vi "Preset_Edit.vi"() -> ()   [LabVIEW 2020, in "Sgraph_lib_V1.lvlib" / "Gviewer.lvclass"]
doc: "Andre Koelewijn, 20 jan 2021\n\nEdit TAGs to display"
uses:
  Gviewer.lvclass
  controls/EditTagOneTag.ctl
  controls/Typedef_Gserver-Replies.ctl
  controls/Typedef_ServerActions.ctl
  DBAL/controls/DBAL_TAGprops.ctl
  DBAL/controls/DBAL_TAGpropEdit.ctl
  Common/controls/typedef_com_TagProp.ctl
  <vilib>/Utility/miscctls.llb/LVPointTypeDef.ctl
  Builds/Sgraph_lib_V1.lvlib
panel:
  in  "PresetPath":path
  in  "PresetName":string
  in  "SaveTime":bool
  in  "OK":bool
  out "tag-info":string
  in  "SaveAs":bool
  in  "Save":bool
  in  "Cancel":bool
  in  "Selector":i32[](listbox)
  in  "Presets":T1[](array[typedef]) {"max" format="%#_3p"; "min" format="%#_3p"}
  in  "Exit_event":bool
  in  "TAGproperties":T2 {"TAGprop"."TagFunc" format="%08x"; "TAGprop"."RangeL" format="%.2f"; "TAGprop"."RangeH" format="%.2f"}
  in  "GViewer-Queue":refnum<queue>
  # "Tag name"
  # "scale L"
  # "scale H"
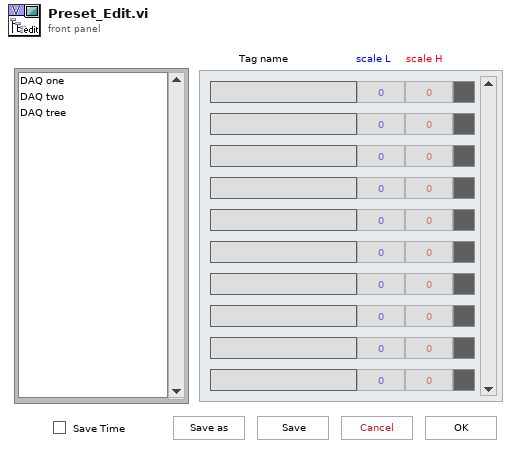
[diagram p1: front panel]
types:
  T1 = typedef "Sgraph_lib_V1.lvlib/Gviewer.lvclass/EditTagOneTag.ctl" = cluster{"TAG":string, "min":dbl, "max":dbl, "Color":u32}
  T2 = typedef "Sgraph_lib_V1.lvlib/DBAL_TAGprops.ctl" = T3[]
  T3 = typedef "Sgraph_lib_V1.lvlib/DBAL_TAGpropEdit.ctl" = cluster{"TAG":string, "Qtype":string, "TAGprop":T4}
  T4 = typedef "Sgraph_lib_V1.lvlib/typedef_com_TagProp.ctl" = cluster{"Description":string, "EngUnits":string, "RangeH":dbl, "RangeL":dbl, "Resolution":i32, "Obsolete":bool, "ChangeDate":timestamp, "ChangeSource":string, "ChangeReason":string, "TagFunc":u32}
  T5 = typedef "LVPointTypeDef.ctl" = cluster{"Horizontal":i16, "Vertical":i16}
  T6 = typedef "Sgraph_lib_V1.lvlib/Typedef_ServerActions.ctl" = enum16{"GraphUpdate", "SendAllTags", "SendIniPath", "SetGeneralOptions", "EditTagsOpen", "EditTagsPresetSave", "EditTagsPresetLoad", "EditTagsClose", "NewTagSelection", "ExitGraph"}
  T7 = typedef "Typedef_Gserver-Replies.ctl" = cluster{"ServerActions":T6, "data":variant, "Source":string, "Time Stamp":timestamp}
  T8 = enum32{"Invalid", "Standard", "Closed", "Hidden", "Minimized", "Maximized"}
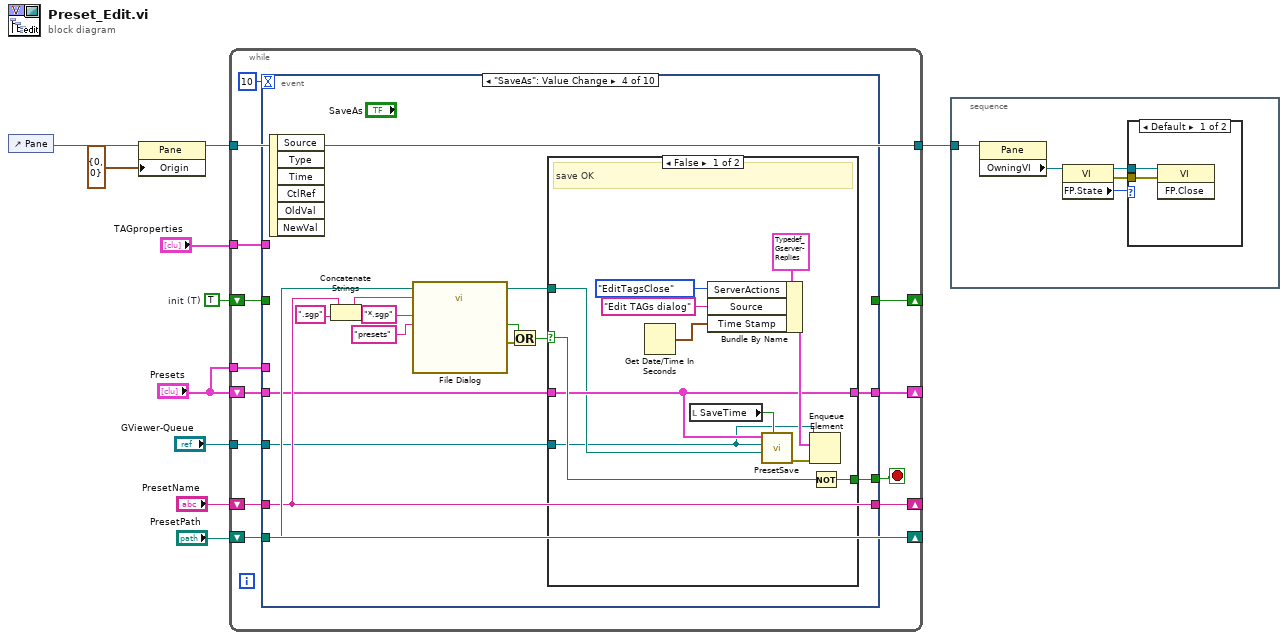
[diagram p0: block diagram]
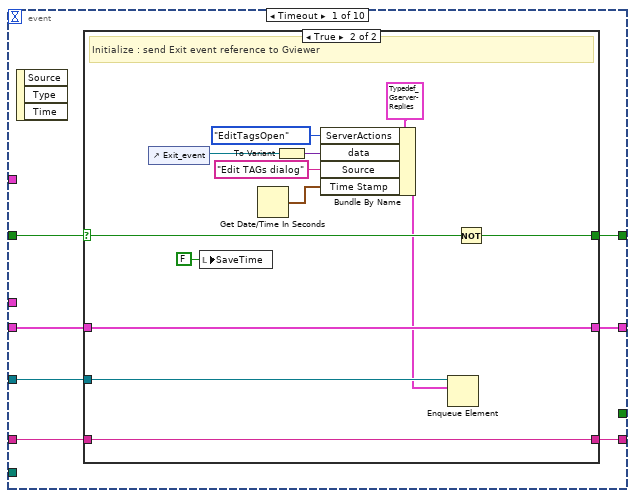
[diagram p3: hidden frame]
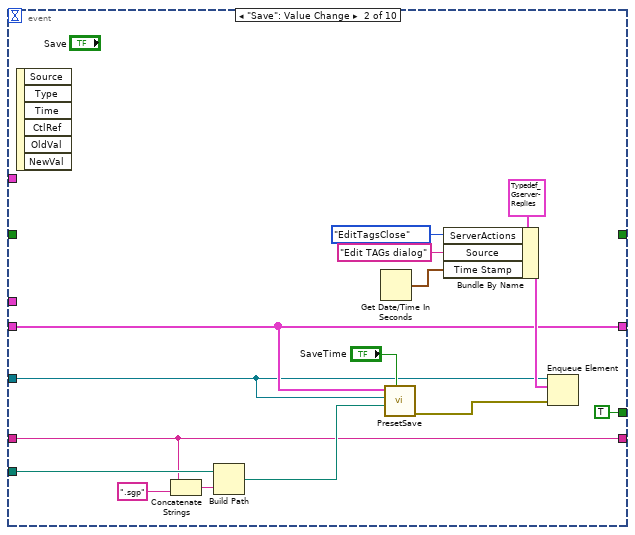
[diagram p5: hidden frame]
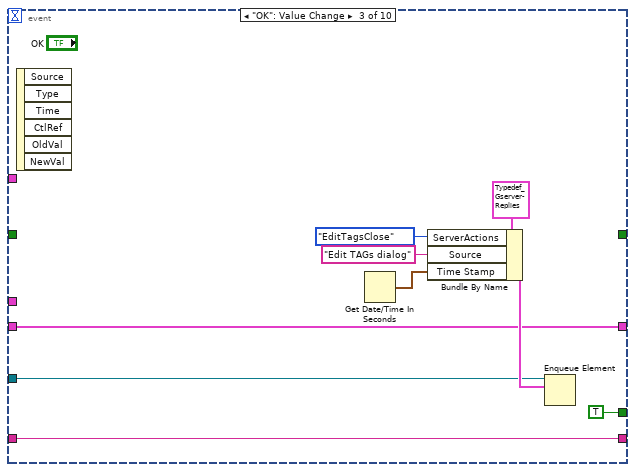
[diagram p6: hidden frame]
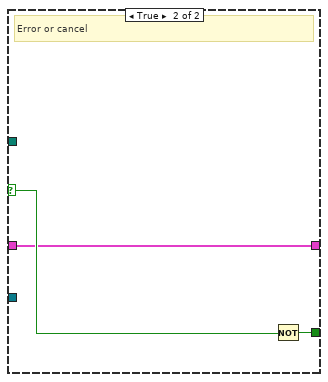
[diagram p7: hidden frame]
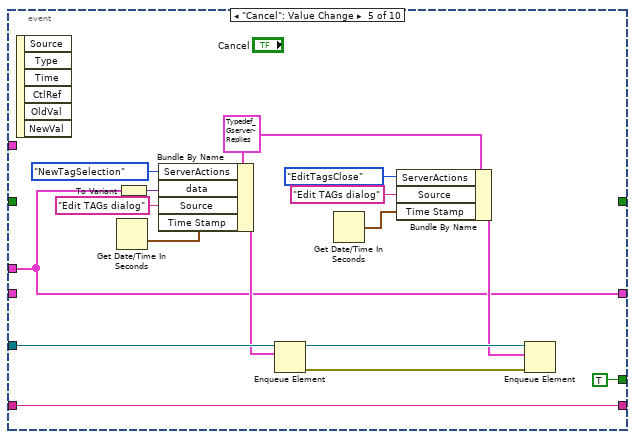
[diagram p8: hidden frame]
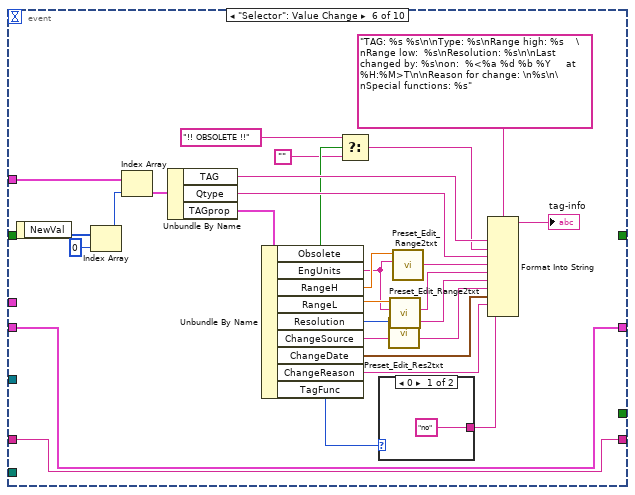
[diagram p9: hidden frame]
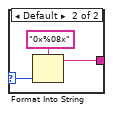
[diagram p10: hidden frame]
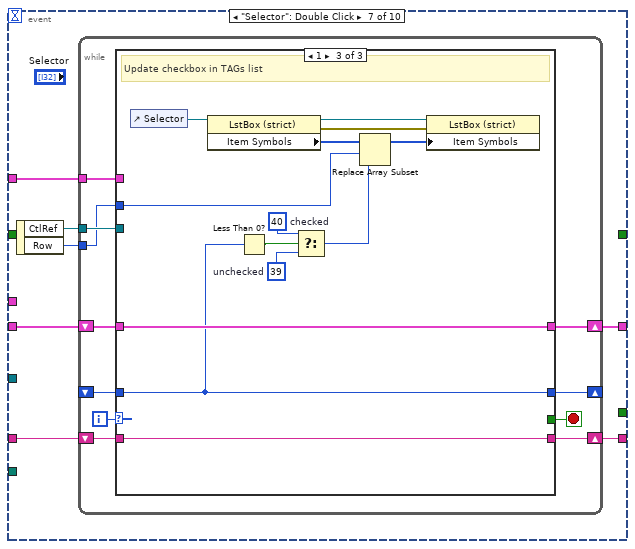
[diagram p11: hidden frame]
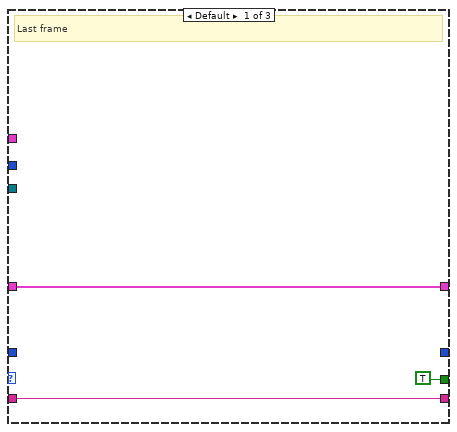
[diagram p12: hidden frame]
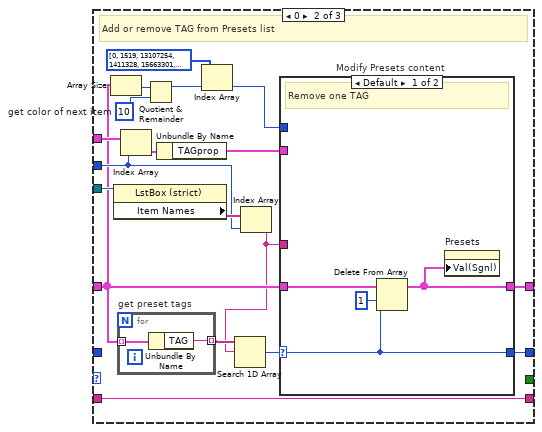
[diagram p13: hidden frame]
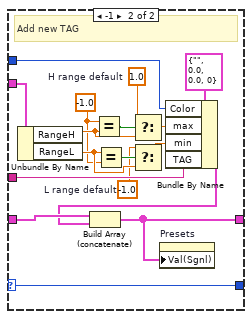
[diagram p14: hidden frame]
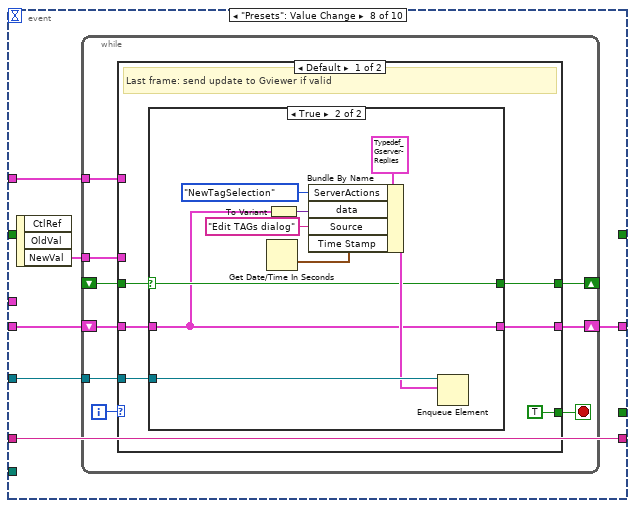
[diagram p15: hidden frame]
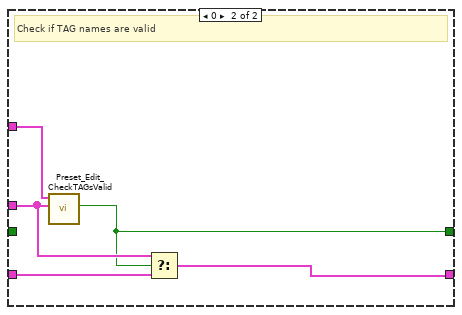
[diagram p17: hidden frame]
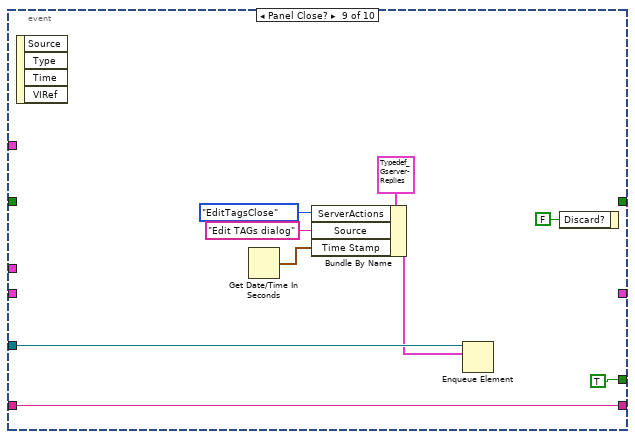
[diagram p18: hidden frame]
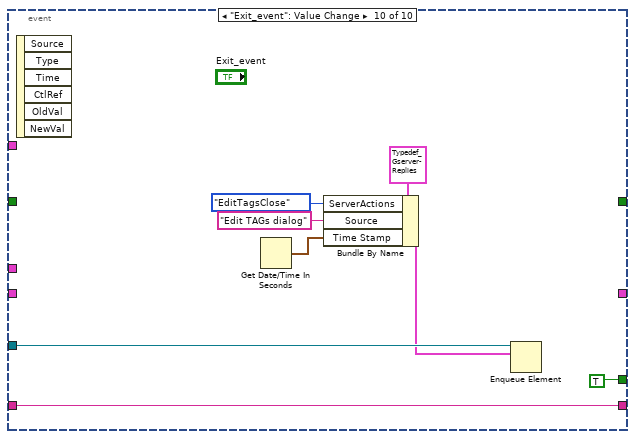
[diagram p19: hidden frame]
diagram:
  w5 = TRUE  # init (T)
  n1 = control-ref of="Pane"() -> (w9:refnum<vi>)
  n2 = property class="Pane"(reference=w9, "Origin"=T5 {"Horizontal"=0, "Vertical"=0}) -> (reference out=w8:refnum<vi>)  [unwired: 1 in, 1 out]
  n3 = while {
    tunnel: w8 -> [w14]
    tunnel: "TAGproperties" -> [w21]
    tunnel: "GViewer-Queue" -> [w18]
    shift-right: [w19] -> _
    shift-left: "Presets" -> [w20]
    shift-right: [w16] -> _
    shift-left: w5 -> [w17]
    tunnel: "Presets" -> [w15]
    tunnel: [w14] -> w3
    shift-right: [w12] -> _
    shift-left: "PresetName" -> [w13]
    shift-right: [w11] -> _
    shift-left: "PresetPath" -> [w11]
    stop <- w23 stop-if-true
    n4 = event shown="[3] \"SaveAs\": Value Change" {
      selector: _ -> [_ _ _ _ _ _ _ _ _ _]
      dyn-events: _ -> [_ _ _ _ _ _ _ _ _ _]
      timeout: 10 -> [_ _ _ _ _ _ _ _ _ _]
      tunnel: [_ TRUE TRUE w75 TRUE _ _ _ TRUE TRUE] -> w23
      tunnel: w21 -> [_ _ _ _ _ w143 w150 w224 _ _]
      tunnel: w20 -> [w29 w51 w64 w73 _ w117 w152 w228 _ _]
      tunnel: [w28 w51 w64 w72 w102 w117 w151 w227 _ _] -> w19
      tunnel: w18 -> [w26 w50 w62 w71 w111 _ _ w226 w262 w275]
      tunnel: w17 -> [w30 _ _ _ _ _ _ _ _ _]
      tunnel: [w27 _ _ _ _ _ _ _ _ _] -> w16
      tunnel: w15 -> [_ _ _ _ w102 _ _ _ _ _]
      tunnel: w13 -> [w25 w48 w63 w81 w100 w116 w149 w223 w260 w269]
      tunnel: [w24 w48 w63 w81 w100 w116 w148 w223 w260 w269] -> w12
      tunnel: w11 -> [_ w49 _ w84 _ _ _ _ _ _]
      event Timeout {
        n5 = event-data() -> ()  [unwired: 1 in, 3 out]
        n6 = case shown="True" w30 {
          selector: w30 -> [w32 w45]
          tunnel: w29 -> [w33 w46]
          tunnel: [w33 w46] -> w28
          tunnel: [w32 w44] -> w27
          tunnel: w26 -> [_ w43]
          tunnel: w25 -> [w31 w34]
          tunnel: [w31 w34] -> w24
          frame False {
            # "normal idle operation"
          }
          frame True {
            # "Initialize : send Exit event reference to Gviewer"
            n7 = control-ref of="Exit_event"() -> (w40:refnum<vi>)
            n8 = local write "SaveTime"(FALSE ("TimeToo")) -> ()
            n9 = Get Date/Time In Seconds() -> (seconds since 1Jan1904=w37:timestamp)
            n10 = To Variant(anything=w40) -> (Variant=w39:variant)
            n11 = Bundle By Name(cluster=T7 {"ServerActions"=enum."GraphUpdate", "data"=variant, "Source"="", "Time Stamp"=timestamp(0 s since 1904-01-01)} ("element"), "ServerActions"=Typedef_ServerActions."EditTagsOpen", "data"=w39, "Source"="Edit TAGs dialog", "Time Stamp"=w37) -> (w36:T7)
            n12 = Enqueue Element(queue=w43, element=w36) -> ()  [unwired: 2 in, 3 out]
            n13 = Not(x=w45) -> (.not. x?=w44:bool)
          }
        }
      }
      event "Save": Value Change {
        n14 = event-data() -> ()  [unwired: 1 in, 6 out]
        n15 = Concatenate Strings(w48, ".sgp" ("string")) -> (w55:string)
        n16 = Build Path(base path=w49, name or relative path=w55) -> (appended path=w54:path)
        n17 = Get Date/Time In Seconds() -> (seconds since 1Jan1904=w61:timestamp)
        n18 = call "PresetSave.vi"("Save time?"="SaveTime", "PresetFilePath"=w54, "GViewer-Queue"=w50, "Presets"=w51) -> ("error out"=w47:errorcluster)  [unwired: 7 in]
        n19 = Bundle By Name(cluster=T7 {"ServerActions"=enum."GraphUpdate", "data"=variant, "Source"="", "Time Stamp"=timestamp(0 s since 1904-01-01)} ("element"), "ServerActions"=Typedef_ServerActions."EditTagsClose", "Source"="Edit TAGs dialog", "Time Stamp"=w61) -> (w60:T7)
        n20 = Enqueue Element(queue=w50, element=w60, error in (no error)=w47) -> ()  [unwired: 1 in, 3 out]
      }
      event "OK": Value Change {
        n21 = event-data() -> ()  [unwired: 1 in, 6 out]
        n22 = Get Date/Time In Seconds() -> (seconds since 1Jan1904=w70:timestamp)
        n23 = Bundle By Name(cluster=T7 {"ServerActions"=enum."GraphUpdate", "data"=variant, "Source"="", "Time Stamp"=timestamp(0 s since 1904-01-01)} ("element"), "ServerActions"=Typedef_ServerActions."EditTagsClose", "Source"="Edit TAGs dialog", "Time Stamp"=w70) -> (w66:T7)
        n24 = Enqueue Element(queue=w62, element=w66) -> ()  [unwired: 2 in, 3 out]
      }
      event "SaveAs": Value Change {
        n25 = event-data() -> ()  [unwired: 1 in, 6 out]
        n26 = Concatenate Strings(w81, ".sgp" ("string")) -> (w80:string)
        n27 = call "File Dialog"("start path"=w84, "default name"=w80, "pattern (all files)"="*.sgp" ("string"), "pattern label"="presets") -> ("selected path"=w74:path, "cancelled"=w77:bool, "error out"=w78:errorcluster)  [unwired: 8 in, 1 out]
        n28 = Or(x=w77, y=w78) -> (x .or. y?=w76:bool)
        n29 = case shown="False" w76 {
          selector: w76 -> [w96 w99]
          tunnel: [w95 w98] -> w75
          tunnel: w74 -> [w86 _]
          tunnel: w73 -> [w87 w97]
          tunnel: [w87 w97] -> w72
          tunnel: w71 -> [w85 _]
          frame False {
            # "save OK"
            n30 = Get Date/Time In Seconds() -> (seconds since 1Jan1904=w93:timestamp)
            n31 = local read "SaveTime"() -> (w91:bool)
            n32 = Bundle By Name(cluster=T7 {"ServerActions"=enum."GraphUpdate", "data"=variant, "Source"="", "Time Stamp"=timestamp(0 s since 1904-01-01)} ("element"), "ServerActions"=Typedef_ServerActions."EditTagsClose", "Source"="Edit TAGs dialog", "Time Stamp"=w93) -> (w94:T7)
            n33 = call "PresetSave.vi"("Save time?"=w91, "PresetFilePath"=w86, "GViewer-Queue"=w85, "Presets"=w87) -> ("error out"=w92:errorcluster)  [unwired: 7 in]
            n34 = Enqueue Element(queue=w85, element=w94, error in (no error)=w92) -> ()  [unwired: 1 in, 3 out]
            n35 = Not(x=w96) -> (.not. x?=w95:bool)
          }
          frame True {
            # "Error or cancel"
            n36 = Not(x=w99) -> (.not. x?=w98:bool)
          }
        }
      }
      event "Cancel": Value Change {
        w106 = T7 {"ServerActions"=enum."GraphUpdate", "data"=variant, "Source"="", "Time Stamp"=timestamp(0 s since 1904-01-01)} ("element")
        n37 = event-data() -> ()  [unwired: 1 in, 6 out]
        n38 = Get Date/Time In Seconds() -> (seconds since 1Jan1904=w115:timestamp)
        n39 = To Variant(anything=w102) -> (Variant=w114:variant)
        n40 = Bundle By Name(cluster=w106, "ServerActions"=Typedef_ServerActions."NewTagSelection", "data"=w114, "Source"="Edit TAGs dialog", "Time Stamp"=w115) -> (w110:T7)
        n41 = Enqueue Element(queue=w111, element=w110) -> (queue out=w104:refnum<queue>, error out=w105:errorcluster)  [unwired: 2 in, 1 out]
        n42 = Get Date/Time In Seconds() -> (seconds since 1Jan1904=w109:timestamp)
        n43 = Bundle By Name(cluster=w106, "ServerActions"=Typedef_ServerActions."EditTagsClose", "Source"="Edit TAGs dialog", "Time Stamp"=w109) -> (w103:T7)
        n44 = Enqueue Element(queue=w104, element=w103, error in (no error)=w105) -> ()  [unwired: 1 in, 3 out]
      }
      event "Selector": Value Change {
        n45 = event-data() -> ("NewVal"=w142:i32[])  [unwired: 1 in]
        n46 = Index Array(array=w142, index=0) -> (element=w140:i32)
        n47 = Index Array(array=w143, index=w140) -> (element=w139:T3)
        n48 = Unbundle By Name(w139) -> ("TAG"=w130:string, "Qtype"=w136:string, "TAGprop"=w138:T4)
        n49 = Unbundle By Name(w138) -> ("Obsolete"=w129:bool, "EngUnits"=w123:string, "RangeH"=w125:dbl, "RangeL"=w124:dbl, "Resolution"=w121:i32, "ChangeSource"=w135:string, "ChangeDate"=w134:timestamp, "ChangeReason"=w133:string, "TagFunc"=w119:u32)
        n50 = Select(t="!! OBSOLETE !!" ("format string"), s=w129, f="") -> (s? t:f=w128:string)
        n51 = case shown="0" w119 {
          selector: w119 -> [_ w146]
          tunnel: ["no" w145] -> w118
          frame 0 {
          }
          frame Default {
            n52 = Format Into String(format string="0x%08x", w146) -> (resulting string=w145:string)  [unwired: 2 in, 1 out]
          }
        }
        n53 = call "Preset_Edit_Res2txt.vi"("Resolution"=w121) -> ("Resolution text"=w120:string)  [unwired: 10 in]
        n54 = call "Preset_Edit_Range2txt.vi"("Engineering units"=w123, "Range"=w124) -> ("RangeInfo"=w122:string)  [unwired: 9 in]
        n55 = call "Preset_Edit_Range2txt.vi"("Engineering units"=w123, "Range"=w125) -> ("RangeInfo"=w126:string)  [unwired: 9 in]
        n56 = Format Into String(format string="TAG: %s %s\n\nType: %s\nRange high: %s    \nRange low:  %s\nResolution: %s\n\nLast changed by: %s\non:  %<%a %d %b %Y     at  %H:%M>T\n\nReason for change: \n%s\n\nSpecial functions: %s", w130, w128, w136, w126, w122, w120, w135, w134, w133, w118) -> (resulting string=→"tag-info":string)  [unwired: 2 in, 1 out]
      }
      event "Selector": Double Click {
        n57 = event-data() -> ("CtlRef"=w154:refnum<vi>, "Row"=w153:i32)  [unwired: 1 in]
        n58 = while {
          tunnel: w154 -> [w161]
          tunnel: w153 -> [w160]
          shift-right: [w163] -> w151
          shift-left: w152 -> [w164]
          tunnel: w150 -> [w162]
          shift-right: [w159] -> _
          shift-left: _ -> [w158]
          shift-right: [w155] -> w148
          shift-left: w149 -> [w156]
          i -> [w165]
          stop <- w157 stop-if-true
          n59 = case shown="1" w165 {
            tunnel: w164 -> [w167 w175 w216]
            tunnel: [w167 w173 w216] -> w163
            tunnel: w162 -> [_ w179 _]
            tunnel: w161 -> [_ w180 _]
            tunnel: w160 -> [_ w178 w217]
            tunnel: [_ w170 w215] -> w159
            tunnel: w158 -> [_ _ w215]
            tunnel: [TRUE _ _] -> w157
            tunnel: w156 -> [w166 w169 w210]
            tunnel: [w166 w169 w210] -> w155
            frame Default {
              # "Last frame"
            }
            frame 0 {
              w185 = 10  # get color of next item
              # "Add or remove TAG from Presets list"
              n60 = Array Size(array=w175) -> (size(s)=w186:i32)
              n61 = property class="LstBox (strict)"(reference=w180) -> ("Item Names"=w182:string[])  [unwired: 1 in, 2 out]
              n62 = for "get preset tags" {
                tunnel: w175 -> [w209] mode=indexing
                tunnel: [w208] -> w177 mode=indexing
                n63 = Unbundle By Name(w209) -> ("TAG"=w208:string)
              }
              n64 = Index Array(array=w179, index=w178) -> (element=w181:T3)
              n65 = Quotient & Remainder(x=w186, y=w185) -> (x-y*floor(x/y)=w183:i32)  [unwired: 1 out]
              n66 = Unbundle By Name(w181) -> ("TAGprop"=w172:T4)
              n67 = Index Array(array=u32[] [0, 1519, 13107254, 1411328, 15663301, 14444288, 40861, 6375227, 6783580, 10450432], index=w183) -> (element=w174:u32)
              n68 = Index Array(array=w182, index=w178) -> (element=w171:string)
              n69 = Search 1D Array(1D array=w177, element=w171) -> (index of element=w176:i32)  [unwired: 1 in]
              n70 = case "Modify Presets content" shown="Default" w176 {
                selector: w176 -> [w188 w192]
                tunnel: [w187 w191] -> w173
                tunnel: w175 -> [w189 w205]
                tunnel: w174 -> [_ w206]
                tunnel: w172 -> [_ w197]
                tunnel: w171 -> [_ w194]
                tunnel: [w188 w192] -> w170
                frame Default {
                  # "Remove one TAG"
                  n71 = Delete From Array(array=w189, length=1, index=w188) -> (array with subset deleted=w187:T1[])  [unwired: 1 out]
                  n72 = property on="Presets" class="Arr (strict)"("Val(Sgnl)"=w187) -> ()  [unwired: 2 in, 2 out]
                }
                frame -1 {
                  w193 = -1.0  # L range default
                  w200 = 1.0  # H range default
                  w199 = -1.0 ("x")
                  # "Add new TAG"
                  n73 = Unbundle By Name(w197) -> ("RangeH"=w204:dbl, "RangeL"=w203:dbl)
                  n74 = Equal?(x=w199, y=w204) -> (x = y?=w201:bool)
                  n75 = Equal?(x=w203, y=w199) -> (x = y?=w202:bool)
                  n76 = Select(t=w200, s=w201, f=w204) -> (s? t:f=w196:dbl)
                  n77 = Select(t=w193, s=w202, f=w203) -> (s? t:f=w195:dbl)
                  n78 = Bundle By Name(cluster=T1 {"TAG"="", "min"=0.0, "max"=0.0, "Color"=0} ("Selected-Tag"), "Color"=w206, "max"=w196, "min"=w195, "TAG"=w194) -> (w198:T1)
                  n79 = Build Array (concatenate)(w205, w198) -> (w191:T1[])
                  n80 = property on="Presets" class="Arr (strict)"("Val(Sgnl)"=w191) -> ()  [unwired: 2 in, 2 out]
                }
              }
            }
            frame 1 {
              w212 = 40  # checked
              w213 = 39  # unchecked
              # "Update checkbox in TAGs list"
              n81 = control-ref of="Selector"() -> (w222:refnum<vi>)
              n82 = property class="LstBox (strict)"(reference=w222) -> (reference out=w221:refnum<vi>, error out=w220:errorcluster, "Item Symbols"=w219:i32[])  [unwired: 1 in]
              n83 = Less Than 0?(x=w215) -> (x < 0?=w214:bool)
              n84 = Select(t=w212, s=w214, f=w213) -> (s? t:f=w211:i32)
              n85 = Replace Array Subset(array=w219, new element=w211, index=w217) -> (w218:i32[])
              n86 = property class="LstBox (strict)"(reference=w221, error in=w220, "Item Symbols"=w218) -> ()  [unwired: 2 out]
            }
          }
        }
      }
      event "Presets": Value Change {
        n87 = event-data() -> ("NewVal"=w225:T1[])  [unwired: 1 in, 2 out]
        n88 = while {
          shift-right: [w235] -> w227
          shift-left: w228 -> [w236]
          tunnel: w226 -> [w233]
          tunnel: w225 -> [w232]
          tunnel: w224 -> [w231]
          shift-right: [w230] -> _
          shift-left: _ -> [w229]
          i -> [w237]
          stop <- w234 stop-if-true
          n89 = case shown="Default" w237 {
            tunnel: w236 -> [w241 w258]
            tunnel: [w238 w256] -> w235
            tunnel: [TRUE _] -> w234
            tunnel: w233 -> [w242 _]
            tunnel: w232 -> [_ w257]
            tunnel: w231 -> [_ w259]
            tunnel: [w239 w255] -> w230
            tunnel: w229 -> [w240 _]
            frame Default {
              # "Last frame: send update to Gviewer if valid"
              n90 = case shown="True" w240 {
                selector: w240 -> [w245 w247]
                tunnel: w242 -> [_ w254]
                tunnel: w241 -> [w244 w246]
                tunnel: [w245 w247] -> w239
                tunnel: [w244 w246] -> w238
                frame False {
                }
                frame True {
                  n91 = Get Date/Time In Seconds() -> (seconds since 1Jan1904=w251:timestamp)
                  n92 = To Variant(anything=w246) -> (Variant=w248:variant)
                  n93 = Bundle By Name(cluster=T7 {"ServerActions"=enum."GraphUpdate", "data"=variant, "Source"="", "Time Stamp"=timestamp(0 s since 1904-01-01)} ("element"), "ServerActions"=Typedef_ServerActions."NewTagSelection", "data"=w248, "Source"="Edit TAGs dialog", "Time Stamp"=w251) -> (w252:T7)
                  n94 = Enqueue Element(queue=w254, element=w252) -> ()  [unwired: 2 in, 3 out]
                }
              }
            }
            frame 0 {
              # "Check if TAG names are valid"
              n95 = call "Preset_Edit_CheckTAGsValid.vi"("Presets-new"=w257, "TAGproperties"=w259) -> ("TAGs OK"=w255:bool)  [unwired: 8 in]
              n96 = Select(t=w257, s=w255, f=w258) -> (s? t:f=w256:T1[])
            }
          }
        }
      }
      event Panel Close? {
        n97 = event-data() -> ()  [unwired: 1 in, 4 out]
        n98 = Get Date/Time In Seconds() -> (seconds since 1Jan1904=w266:timestamp)
        n99 = Bundle By Name(cluster=T7 {"ServerActions"=enum."GraphUpdate", "data"=variant, "Source"="", "Time Stamp"=timestamp(0 s since 1904-01-01)} ("element"), "ServerActions"=Typedef_ServerActions."EditTagsClose", "Source"="Edit TAGs dialog", "Time Stamp"=w266) -> (w261:T7)
        n100 = Enqueue Element(queue=w262, element=w261) -> ()  [unwired: 2 in, 3 out]
        n101 = event-data("Discard?"=FALSE) -> ()  [unwired: 1 in, 1 out]
      }
      event "Exit_event": Value Change {
        n102 = event-data() -> ()  [unwired: 1 in, 6 out]
        n103 = Get Date/Time In Seconds() -> (seconds since 1Jan1904=w272:timestamp)
        n104 = Bundle By Name(cluster=T7 {"ServerActions"=enum."GraphUpdate", "data"=variant, "Source"="", "Time Stamp"=timestamp(0 s since 1904-01-01)} ("element"), "ServerActions"=Typedef_ServerActions."EditTagsClose", "Source"="Edit TAGs dialog", "Time Stamp"=w272) -> (w270:T7)
        n105 = Enqueue Element(queue=w275, element=w270) -> ()  [unwired: 2 in, 3 out]
      }
    }
  }
  n106 = stacked-sequence {
    tunnel: w3 -> [w281]
    frame #0 {
      n107 = property class="Pane"(reference=w281) -> ("OwningVI"=w280:refnum<vi>)  [unwired: 1 in, 2 out]
      n108 = property class="VI"(reference=w280) -> (reference out=w278:refnum<vi>, error out=w277:errorcluster, "FP.State"=w279:T8)  [unwired: 1 in]
      n109 = case shown="Default" w279 {
        tunnel: w278 -> [w283 _]
        tunnel: w277 -> [w282 _]
        frame Default {
          n110 = invoke class="VI" method="FP.Close"(reference=w283, error in=w282) -> ()  [unwired: 1 in, 3 out]
        }
        frame "Closed" {
        }
      }
    }
  }
